vi "shearview_v1_0_oscillatoryshear__bfb7da842b.vi"() -> ()   [LabVIEW 2023]
uses:
  <instrlib>/niDCPower/nidcpower.llb/niDCPower Output Function.ctl
  <instrlib>/niDCPower/nidcpower.llb/niDCPower Source Mode.ctl
  <vilib>/Platform/TimedLoop/XDataNode/nitl_modes.ctl
  <vilib>/Platform/TimedLoop/XDataNode/timing_clust.ctl
  <vilib>/Platform/TimedLoop/XDataNode/wakeup.ctl
  <vilib>/Analysis/1siggen.llb/Ramp Pattern by Samples.vi
  <vilib>/DAQmx/create/channels.llb/DAQmx Create Channel (AI-Voltage-Basic).vi
  <vilib>/platform/TimedLoop/XDataNode/XDataNode.xnode
  <vilib>/Platform/TimedLoop/XDataNode/XDNodeRunTimeDep.lvlib
  <vilib>/Analysis/NI_AALBase.lvlib
panel:
  in  "stop 2":bool
  out "CPU Usage (%)":sgl(slide) scale=0.0..100.0
  out "Processor History":sgl(graph)
  in  "Tab Control 2":T1(tab)
  in  "Title of experiment":string="Shear Profiles " caption="A"
  in  "User":string="Nikos" caption="A"
  in  "Keywords":string caption="A"
  in  "Description":string="Profiles" caption="A"
  in  "Sample":string caption="A"
  in  "Temperature (oC)":string="23" caption="A"
  in  "Objective:":string="ELWD x20 " caption="A"
  in  "Numerical Aperture":string="0.45" caption="A"
  in  "Phase Annulus":string="Ph 1" caption="A"
  in  "Camera":string="Ximea MC050MG-SY-UB" caption="A"
  in  "Binning":string="2x2" caption="A"
  in  "Frame Rate (fps)":string="100 " caption="A"
  out "Finished Late? [i-1]":bool
  out "Iteration Duration":i64 format="%.2f"
  in  "Gap (mm)":dbl=1.0
  in  "Initial position in Voltage (V)":dbl=3.8
  in  "Voltage to Displacement Constant (V/mm)":dbl=0.689
  in  "Strain (%)":dbl=100.0
  in  "Frequency (Hz)":dbl=1.0 format="%0.3f"
  out "Elapsedf time (s)":dbl
  in  "samples":i32=7
  in  "end":dbl=100.0 format="%0.2f"
  in  "start":dbl=10.0 format="%0.2f"
  out "Ramp Pattern":dbl[](array[numeric])
  in  "type":u16(ring)=1 items=["Linear", "Logarithmic"]
  out "amplitude":dbl
  out "PID called time (s)":dbl format="%.3f"
  in  "Initial PID gains":T2={"proportional gain (Kc)"=0.1, "integral time (Ti, min)"=0.01, "derivative time (Td, min)"=0.0} {"derivative time (Td, min)" format="%.5f"; "integral time (Ti, min)" format="%.5f"; "proportional gain (Kc)" format="%.3f"}
  in  "PID dt (s)":dbl=0.003 format="%.3f"
  in  "Output current limit":dbl(slide)=0.49999999999999994 scale=0.0..1.0
  in  "Propotional":dbl(slide)=0.3411214953271028 scale=0.0..1.0
  in  "Integral":dbl(slide)=0.0002102803738317757 scale=0.0..0.0002
  in  "Derivative":dbl(slide) scale=0.0..0.001
  out "task done?":bool
  out "mean strain (-)":dbl
  out "min strain (-)":dbl
  out "max strain (-)":dbl
  out "mean current(A)":dbl
  in  "frames/period":dbl=12.0
  in  "offset (sec)":dbl=0.005
  in  "Exposure (s)  2":dbl=0.0001
  in  "Frequency":dbl=100.0 format="%.6f"
  in  "Duty Cycle":dbl=0.01 format="%.6f"
  in  "Number of Pulses":i32=1000
  in  "Imaging Selection":enum16{"No Imaging", "Profiles", "Echoes"}(ring)
  out "output array":cluster{dbl, dbl}[](array[cluster])
  out "error out":errorcluster
  out "Error":errorcluster
  out "error out 2":errorcluster
  in  "Tab Control":enum32{"Lissajous", "Strain-Stress"}(tab)
  out "?":cluster{dbl[], dbl[]}(graph)
  out "Mixed Signal Graph 5":dynamicdata(graph) caption="Commanded and Actual Strain vs Current"
  out "Queue timed out?":bool
  in  "stop":bool
  in  "stop initial loop":bool
  in  "file path":path=path "C:/Users/PC/Desktop/Data/tests/test.txt"
  # "Control Loop"
  # "Control Loop  Output"
  # "Parameters of Echoes"
  # "Parameters of Profiles"
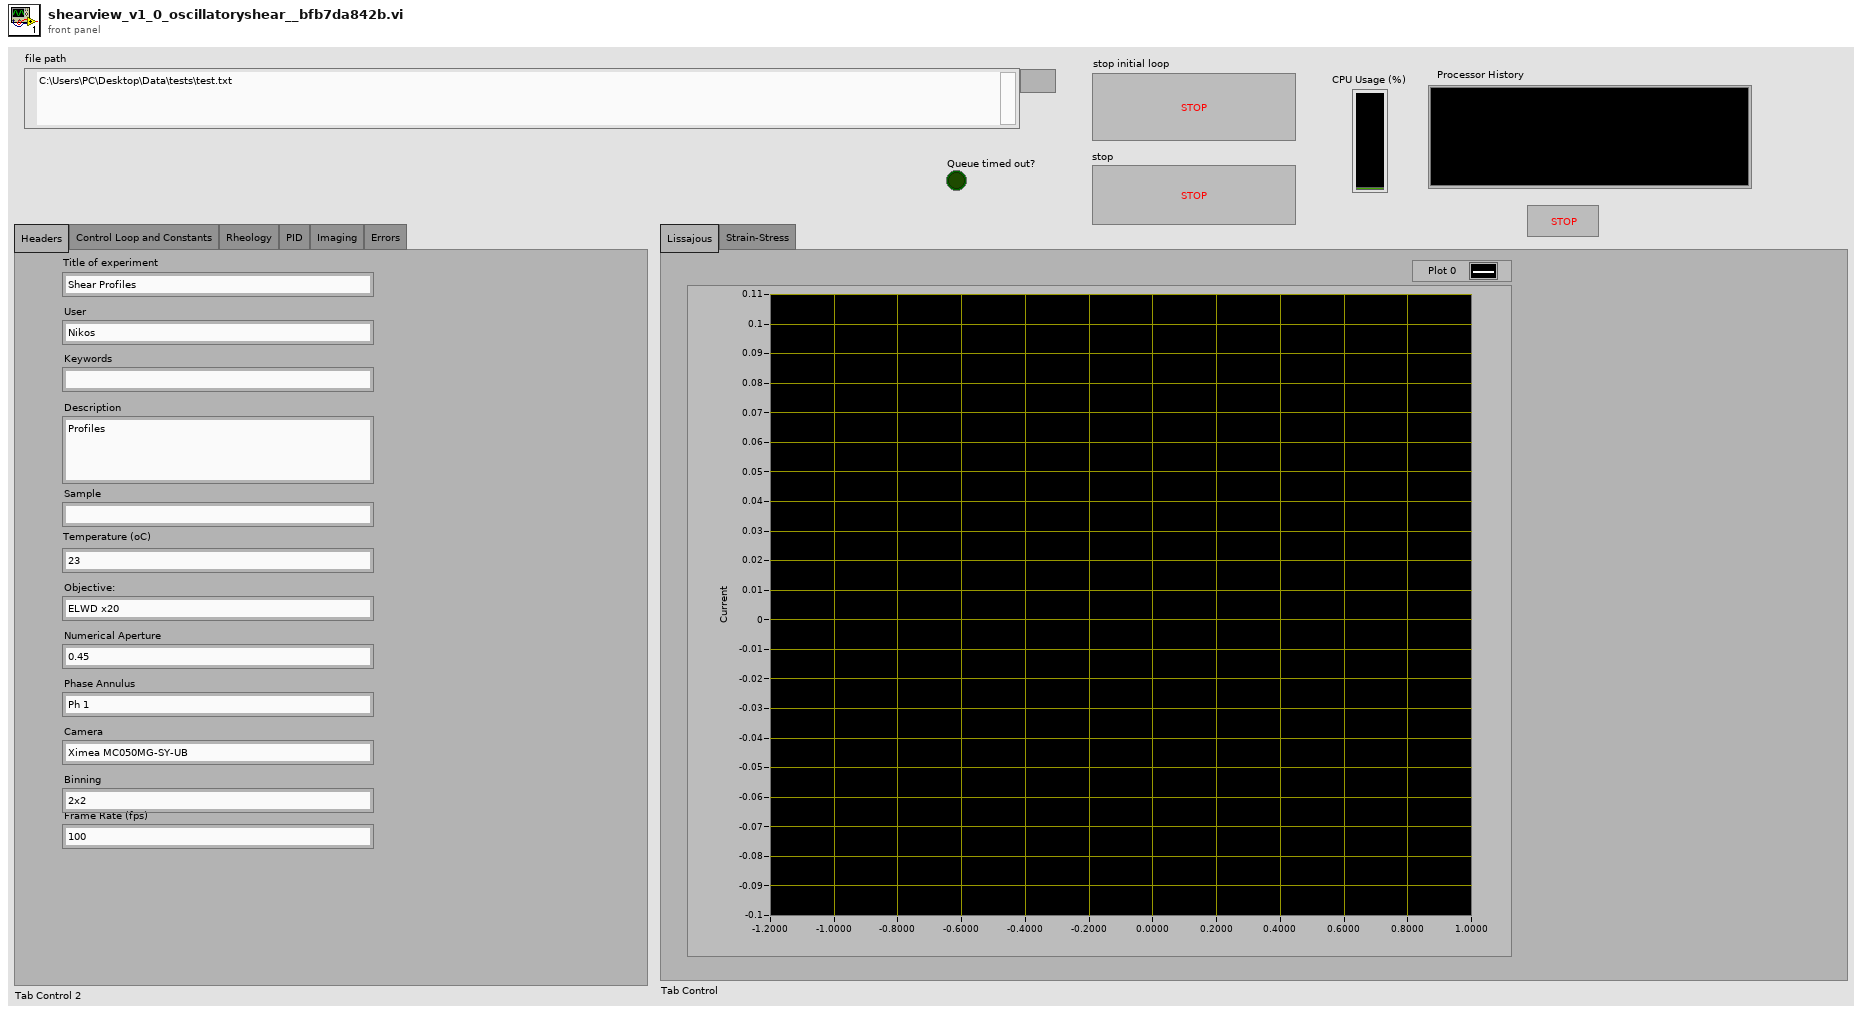
[diagram p1: front panel]
types:
  T1 = enum32{"Headers", "Control Loop and Constants", "Rheology", "PID", "Imaging", "Errors"}
  T2 = cluster{"proportional gain (Kc)":dbl, "integral time (Ti, min)":dbl, "derivative time (Td, min)":dbl}
  T3 = typedef "niDCPower Source Mode.ctl" = i32
  T4 = typedef "niDCPower Output Function.ctl" = i32
  T5 = typedef "XDNodeRunTimeDep.lvlib/nitl_modes.ctl" = enum32{"No Change", "Process missed periods, maintain original phase", "Discard missed periods, maintain original phase", "Process missed periods, ignore original phase", "Discard missed periods, ignore original phase"}
  T6 = typedef "XDNodeRunTimeDep.lvlib/timing_clust.ctl" = cluster{"Expected End [f-1]":u64, "Actual End [f-1]":u64, "Finished Late? [f-1]":bool, "Expected End [i-1]":u64, "Actual End [i-1]":u64, "Finished Late? [i-1]":bool, "Expected Start [i]":u64, "Actual Start [i]":u64, "Expected Start [f]":u64, "Actual Start [f]":u64, "Source Name":string, "Structure Name":string, "Period":i64, "Deadline":i64, "Offset":i64, "Start":i64, "Priority":i32, "Timeout":i32, "Mode":T5, "Wakeup Reason":T7, "Error":errorcluster, "Source Type":string, "Secondary Source Type":string, "Global End Time":u64, "Global Start Time":u64, "Frame Duration":u64, "Iteration Duration":u64, "Assigned CPU":i32, "I/O Scan Engine Mode":u32}
  T7 = typedef "XDNodeRunTimeDep.lvlib/wakeup.ctl" = enum32{"Normal", "Aborted", "Asynchronous wakeup", "Timing source error", "Timed loop error", "Timeout"}
  T8 = cluster{"time":dbl, "data":dbl, "set point":dbl, "time stress":dbl, "voltage":dbl, "current":dbl}
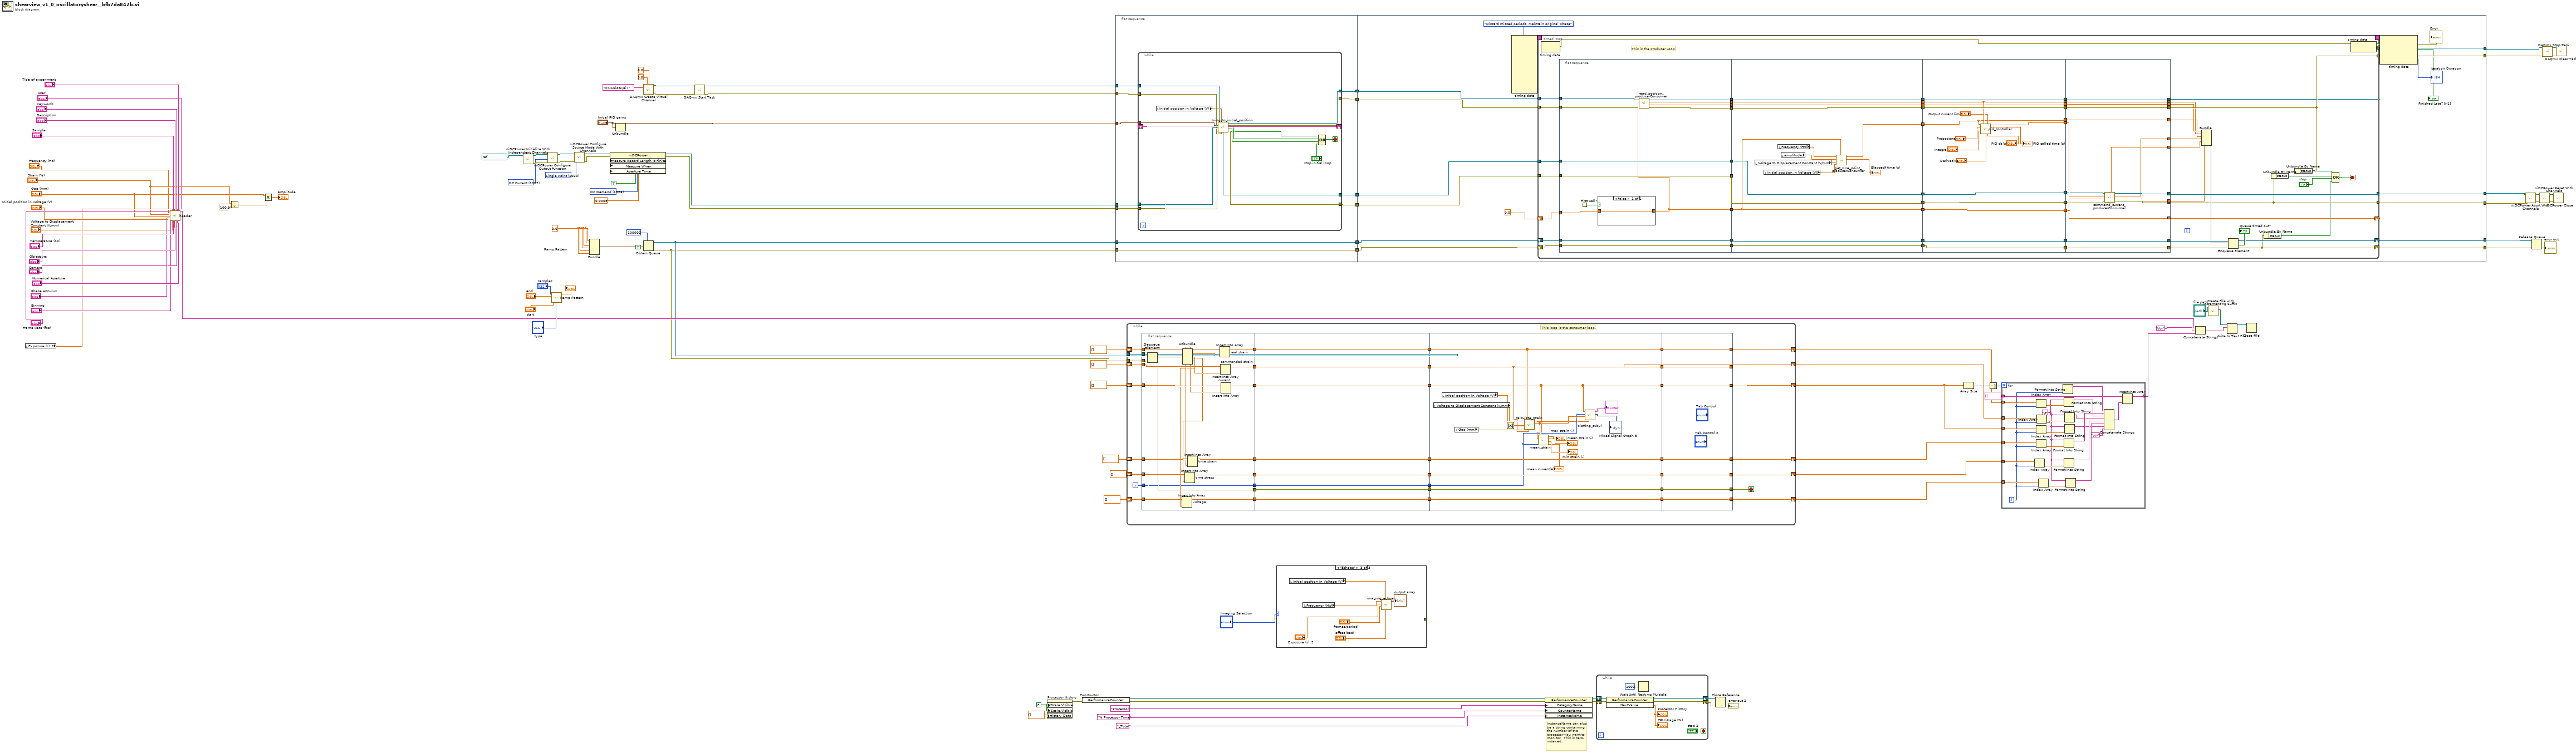
[diagram p0: block diagram]
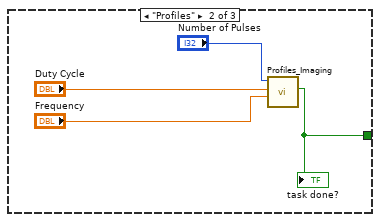
[diagram p3: hidden frame]
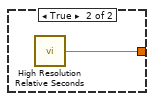
[diagram p4: hidden frame]
diagram:
  w7 = FALSE ("X Scale.Visible")
  w27 = 0.0
  w65 = T3 1020 items=["Single Point"=1020, "Sequence"=1021] ("source mode")
  w95 = 1026 items=["Automatically after Source Complete"=1025, "On Demand"=1026, "On Measure Trigger"=1027] ("Measurement:Advanced:Measure When")
  w101 = T4 1007 items=["DC Voltage"=1006, "DC Current"=1007, "Pulse Voltage"=1049, "Pulse Current"=1050] ("output function")
  # "InstanceName can also\nbe a string containing\nthe number of the\nprocessor you want to\nmonitor.  This is zero-\nindexed."
  n1 = local read "Exposure (s)  2"() -> (w45:dbl)
  n2 = call "header.vi"("Frequency (Hz)"="Frequency (Hz)", "Frame Rate (fps)"="Frame Rate (fps)", "Strain (%)"="Strain (%)", "Binning"="Binning", "Gap (mm)"="Gap (mm)", "Phase Annulus"="Phase Annulus", "Initial position in Voltage (V)"="Initial position in Voltage (V)", "Exposure (s)"=w45, "Voltage to Displacement Constant (V/mm)"="Voltage to Displacement Constant (V/mm)", "Sample"="Sample", "Temperature (oC)"="Temperature (oC)", "Description"="Description", "Objective:"="Objective:", "Keywords"="Keywords", "Camera"="Camera", "User"="User", "Numerical Aperture"="Numerical Aperture", "Title of experiment"="Title of experiment") -> ("String"=w44:string)  [unwired: 9 in]
  n3 = Divide(x="Strain (%)", y=100.0) -> (x/y=w43:dbl)
  n4 = Multiply(x="Gap (mm)", y=w43) -> (x*y=→"amplitude":dbl)
  n5 = call <instrlib>:"niDCPower Initialize With Independent Channels.vi"("resource name"=refnum<k15> "PXI1Slot3") -> ("error out"=w103:errorcluster, "instrument handle out"=w102:refnum<k15>)  [unwired: 9 in]
  n6 = call <instrlib>:"niDCPower Configure Output Function.vi"("error in (no error)"=w103, "output function"=w101, "instrument handle"=w102) -> ("error out"=w99:errorcluster, "instrument handle out"=w100:refnum<k15>)  [unwired: 7 in]
  n7 = call-poly <vilib>:"Ramp Pattern.vi"("type"="type", "start"="start", "end"="end", "samples"="samples") -> ("Ramp Pattern"=→"Ramp Pattern":dbl[])  [unwired: 6 in, 1 out]
  n8 = call <instrlib>:"niDCPower Configure Source Mode With Channels.vi"("error in (no error)"=w99, "source mode"=w65, "instrument handle"=w100) -> ("error out"=w91:errorcluster, "instrument handle out"=w90:refnum<k15>)  [unwired: 7 in]
  n9 = Bundle(w27, w27, w27, w27, w27, w27) -> (w28:cluster{dbl, dbl, dbl, dbl, dbl, dbl})  [unwired: 1 in]
  n10 = property class="niDCPower"(reference=w90, error in=w91, "Measure Record Length Is Finite"=TRUE ("Measurement:Measure Record Length Is Finite"), "Measure When"=w95, "Aperture Time"=0.0005 ("Measurement:Aperture Time")) -> (reference out=w73:refnum<k15>, error out=w94:errorcluster)
  n11 = Unbundle("Initial PID gains") -> ()  [unwired: 3 out]
  n12 = Obtain Queue(max queue size (-1, unlimited)=100000, element data type=w28, create if not found? (T)=TRUE) -> (queue out=w18:refnum<queue>, error out=w17:errorcluster)  [unwired: 2 in, 1 out]
  n13 = call-poly <vilib>:"DAQmx Create Virtual Channel.vi"("maximum value"=5.0, "minimum value"=0.0, "physical channels"=tag "PXI1Slot2/ai7") -> ("task out"=w86:refnum<k21>, "error out"=w85:errorcluster)  [unwired: 11 in]
  n14 = call <vilib>:"DAQmx Start Task.vi"("task/channels in"=w86, "error in"=w85) -> ("task out"=w106:refnum<k21>, "error out"=w66:errorcluster)  [unwired: 12 in]
  n15 = property on="Processor History" class="WFChart (strict)"("XScale.Visible"=w7, "YScale.Visible"=w7, "History Data"=sgl[] []) -> (error out=w4:errorcluster)  [unwired: 2 in, 1 out]
  n16 = constructor class="PerformanceCounter" ("Constructor Node")(error in=w4) -> (reference out=w16:refnum<k24>, error out=w15:errorcluster)  [unwired: 2 in, 1 out]
  n17 = flat-sequence {
    tunnel: w94 -> [w119]
    tunnel: w73 -> [w120]
    tunnel: w106 -> [w113]
    tunnel: [w117] -> w93
    tunnel: [w118] -> w92
    tunnel: "Initial PID gains" -> [w112]
    tunnel: [w116] -> w75
    tunnel: [w115] -> w74
    tunnel: w66 -> [w114]
    tunnel: [w111] -> w24
    tunnel: w18 -> [w111]
    tunnel: [w110] -> w23
    tunnel: w17 -> [w110]
    tunnel: [w154] -> w97
    tunnel: [w153] -> w3
    tunnel: w92 -> [w155]
    tunnel: w93 -> [w156]
    tunnel: [w138] -> w80
    tunnel: [w147] -> w79
    tunnel: w75 -> [w146]
    tunnel: w74 -> [w145]
    tunnel: [w142] -> w64
    tunnel: [w143] -> w63
    tunnel: w24 -> [w141]
    tunnel: w23 -> [w140]
    frame #0 {
      n18 = while {
        tunnel: [w137] -> w116
        tunnel: [w134] -> w115
        tunnel: w120 -> [w136]
        tunnel: w119 -> [w135]
        tunnel: [w133] -> w117
        tunnel: w113 -> [w124]
        tunnel: w114 -> [w123]
        tunnel: [w132] -> w118
        shift-right: [w131] -> _
        shift-left: _ -> [w130]
        tunnel: w112 -> [w122]
        stop <- w126 stop-if-true
        n19 = local read "Initial position in Voltage (V)"() -> (w121:dbl)
        n20 = call "bring_to_initial_position.vi"("Refnum in"=w124, "Initial position in Voltage (V) in"=w121, "Initial PID gains"=w122, "instrument handle in"=w136, "Array in"=w130, "error in (no error)"=w135, "error in"=w123) -> ("instrument handle out"=w132:refnum<k15>, "status"=w127:bool, "Refnum out"=w137:refnum<k21>, "error out 3"=w134:errorcluster, "status 2"=w128:bool, "Boolean"=w129:bool, "Array out"=w131:string[], "error out"=w133:errorcluster)  [unwired: 1 in]
        n21 = Compound Arithmetic op=OR(w127, w128, w129, "stop initial loop") -> (w126:bool)
      }
    }
    frame #1 {
      n22 = node-c288(nitl_modes."Discard missed periods, maintain original phase" ("Mode")) -> (w152:T6)  [unwired: 9 in]
      n23 = timed-loop {
        tunnel: w156 -> [w193]
        shift-right: [w177] -> _
        shift-left: 0.0 ("relative seconds") -> [w209]
        tunnel: w146 -> [w202]
        tunnel: w145 -> [w201]
        tunnel: w155 -> [w197]
        tunnel: [w191] -> w154
        tunnel: [w192] -> w153
        tunnel: [w189] -> w147
        timing: w152 -> [_]
        timing-out: [_] -> w151
        shift-right: [w161] -> w142
        shift-left: w141 -> [w184]
        shift-right: [w160] -> w143
        shift-left: w140 -> [w163]
        tunnel: [w157] -> w138
        stop <- w158 stop-if-true
        # "This is the Producer Loop"
        n24 = node-c288() -> (w188:errorcluster)  [unwired: 1 in]
        n25 = flat-sequence {
          tunnel: w202 -> [w232]
          tunnel: [w229] -> w216
          tunnel: [w234] -> w214
          tunnel: [w233] -> w211
          tunnel: w209 -> [w228]
          tunnel: w201 -> [w226]
          tunnel: [w231] -> w198
          tunnel: w197 -> [w231]
          tunnel: [w230] -> w194
          tunnel: w193 -> [w230]
          tunnel: [w227] -> w190
          tunnel: w184 -> [w224]
          tunnel: [w224] -> w183
          tunnel: [w223] -> w176
          tunnel: [w222] -> w164
          tunnel: w163 -> [w222]
          tunnel: w216 -> [w251]
          tunnel: [w251] -> w215
          tunnel: w214 -> [w250]
          tunnel: [w250] -> w213
          tunnel: [w247] -> w212
          tunnel: w211 -> [w248]
          tunnel: [w248] -> w210
          tunnel: [w237] -> w208
          tunnel: [w249] -> w199
          tunnel: w198 -> [w249]
          tunnel: [w245] -> w195
          tunnel: w194 -> [w245]
          tunnel: w190 -> [w237]
          tunnel: w183 -> [w244]
          tunnel: [w244] -> w181
          tunnel: w176 -> [w243]
          tunnel: [w243] -> w175
          tunnel: w164 -> [w238]
          tunnel: [w238] -> w162
          tunnel: w215 -> [w264]
          tunnel: w213 -> [w268]
          tunnel: w212 -> [w253]
          tunnel: w210 -> [w263]
          tunnel: w208 -> [w267]
          tunnel: [w264] -> w207
          tunnel: [w268] -> w206
          tunnel: [w263] -> w205
          tunnel: [w256] -> w204
          tunnel: [w267] -> w203
          tunnel: [w265] -> w200
          tunnel: w199 -> [w265]
          tunnel: [w266] -> w196
          tunnel: w195 -> [w266]
          tunnel: [w255] -> w182
          tunnel: w181 -> [w255]
          tunnel: [w252] -> w178
          tunnel: w175 -> [w254]
          tunnel: [w254] -> w174
          tunnel: [w253] -> w172
          tunnel: w162 -> [w252]
          tunnel: [w278] -> w177
          tunnel: [w282] -> w167
          tunnel: [w283] -> w192
          tunnel: [w284] -> w191
          tunnel: w207 -> [w284]
          tunnel: w206 -> [w283]
          tunnel: w205 -> [w282]
          tunnel: w204 -> [w281]
          tunnel: w203 -> [w278]
          tunnel: w200 -> [w277]
          tunnel: w196 -> [w280]
          tunnel: [w279] -> w157
          tunnel: [w276] -> w189
          tunnel: [w275] -> w180
          tunnel: w182 -> [w275]
          tunnel: [w274] -> w179
          tunnel: w178 -> [w274]
          tunnel: w174 -> [w273]
          tunnel: [w273] -> w173
          tunnel: [w272] -> w166
          tunnel: w172 -> [w272]
          tunnel: [w271] -> w171
          tunnel: [w270] -> w170
          tunnel: [w269] -> w169
          frame #0 {
            n26 = First Call?() -> (First Call?: T/F=w225:bool)
            n27 = case shown="False" w225 {
              tunnel: [w235 w236] -> w227
              tunnel: w228 -> [w235 _]
              frame False {
              }
              frame True {
                n28 = call <vilib>:"High Resolution Relative Seconds.vi"() -> ("relative seconds"=w236:dbl)
              }
            }
            n29 = call "read_position_producerConsumer.vi"("error in (no error)"=w226, "relative seconds"=w227, "Refnum in"=w232) -> ("error out"=w234:errorcluster, "time"=w223:dbl, "data"=w233:dbl, "Refnum out"=w229:refnum<k21>)  [unwired: 5 in]
          }
          frame #1 {
            n30 = local read "Voltage to Displacement Constant (V/mm)"() -> (w240:dbl)
            n31 = local read "Initial position in Voltage (V)"() -> (w239:dbl)
            n32 = local read "Frequency (Hz)"() -> (w242:dbl)
            n33 = local read "amplitude"() -> (w241:dbl)
            n34 = call "get_sine_point_producerConsumer.vi"("relative seconds"=w237, "Initial position in voltage"=w239, "voltage to displacement constant"=w240, "amplitude"=w241, "frequency"=w242) -> ("Elapsedf time (s)"=→"Elapsedf time (s)":dbl, "set point"=w247:dbl)  [unwired: 5 in]
          }
          frame #2 {
            n35 = call "pid_controller.vi"("set point"=w253, "process variable"=w263, "Output current limit"="Output current limit", "Propotional"="Propotional", "Integral"="Integral", "Derivative"="Derivative", "PID dt (s)"="PID dt (s)") -> ("output"=w256:dbl, "PID called time (s)"=→"PID called time (s)":dbl)  [unwired: 7 in]
          }
          frame #3 {
            n36 = call "command_current_producerConsumer.vi"("error in (no error)"=w280, "relative seconds"=w278, "PID output"=w281, "IVI Refnum in"=w277) -> ("error out"=w279:errorcluster, "time stress"=w271:dbl, "IVI Refnum out"=w276:refnum<k15>, "current"=w269:dbl, "voltage"=w270:dbl)  [unwired: 3 in]
          }
        }
        n37 = Bundle("time"=w173, "data"=w167, "set point"=w166, "time stress"=w171, "voltage"=w170, "current"=w169) -> (w168:T8)  [unwired: 1 in]
        n38 = Enqueue Element(queue=w180, element=w168, error in (no error)=w179) -> (queue out=w161:refnum<queue>, timed out?=→"Queue timed out?":bool, error out=w160:errorcluster)  [unwired: 1 in]
        n39 = Unbundle By Name(w160) -> ("status"=w159:bool)
        n40 = Unbundle By Name(w157) -> ("status"=w186:bool)
        n41 = Unbundle By Name(w192) -> ("status"=w187:bool)
        n42 = Compound Arithmetic op=OR(w187, w186, "stop", w159) -> (w158:bool)
        n43 = node-c288(w188) -> ()  [unwired: 1 out]
      }
      n44 = node-c288(w151) -> (→"Error":errorcluster, →"Finished Late? [i-1]":bool, →"Iteration Duration":i64)  [unwired: 1 out]
    }
  }
  n45 = while {
    tunnel: w18 -> [w330]
    shift-right: [w328] -> w22
    shift-left: dbl[] [] -> [w329]
    shift-right: [w327] -> w34
    shift-left: dbl[] [] -> [w326]
    shift-right: [w325] -> w33
    shift-left: dbl[] [] -> [w324]
    shift-right: [w322] -> w35
    shift-left: dbl[] [] -> [w323]
    shift-right: [w319] -> w31
    shift-left: dbl[] [] -> [w320]
    shift-right: [w321] -> w32
    shift-left: dbl[] [] -> [w318]
    tunnel: w17 -> [w317]
    i -> [w293]
    stop <- w296 stop-if-true
    # "This loop is the consumer loop."
    n46 = flat-sequence {
      tunnel: w330 -> [w353]
      tunnel: w329 -> [w351]
      tunnel: w326 -> [w348]
      tunnel: w324 -> [w346]
      tunnel: w323 -> [w345]
      tunnel: w320 -> [w342]
      tunnel: w318 -> [w340]
      tunnel: w317 -> [w339]
      tunnel: [w350] -> w316
      tunnel: [w349] -> w315
      tunnel: [w347] -> w314
      tunnel: [w344] -> w313
      tunnel: [w343] -> w312
      tunnel: [w341] -> w311
      tunnel: [w332] -> w298
      tunnel: [w331] -> w294
      tunnel: w293 -> [w331]
      tunnel: w316 -> [w361]
      tunnel: w315 -> [w360]
      tunnel: w314 -> [w359]
      tunnel: w313 -> [w358]
      tunnel: w312 -> [w357]
      tunnel: w311 -> [w356]
      tunnel: [w361] -> w310
      tunnel: [w360] -> w309
      tunnel: [w359] -> w308
      tunnel: [w358] -> w307
      tunnel: [w357] -> w306
      tunnel: [w356] -> w305
      tunnel: w298 -> [w355]
      tunnel: [w355] -> w297
      tunnel: w294 -> [w354]
      tunnel: [w354] -> w292
      tunnel: w310 -> [w367]
      tunnel: w309 -> [w366]
      tunnel: w308 -> [w362]
      tunnel: w307 -> [w381]
      tunnel: w306 -> [w380]
      tunnel: w305 -> [w379]
      tunnel: [w367] -> w304
      tunnel: [w366] -> w303
      tunnel: [w362] -> w302
      tunnel: [w381] -> w301
      tunnel: [w380] -> w300
      tunnel: [w379] -> w299
      tunnel: w297 -> [w368]
      tunnel: [w368] -> w295
      tunnel: w292 -> [w365]
      tunnel: [w383] -> w319
      tunnel: [w384] -> w321
      tunnel: [w385] -> w322
      tunnel: [w386] -> w325
      tunnel: [w387] -> w327
      tunnel: [w388] -> w328
      tunnel: w304 -> [w388]
      tunnel: w303 -> [w387]
      tunnel: w302 -> [w386]
      tunnel: w301 -> [w385]
      tunnel: w300 -> [w384]
      tunnel: w299 -> [w383]
      tunnel: [w382] -> w296
      tunnel: w295 -> [w382]
      frame #0 {
        n47 = Dequeue Element(queue=w353, error in (no error)=w339) -> (element=w352:cluster{dbl, dbl, dbl, dbl, dbl, dbl}, error out=w332:errorcluster)  [unwired: 1 in, 2 out]
        n48 = Unbundle(w352) -> (w335:dbl, w338:dbl, w337:dbl, w334:dbl, w333:dbl, w336:dbl)
        n49 = Insert Into Array "voltage"(array=w342, new element=w333) -> (w341:dbl[])  [unwired: 1 in]
        n50 = Insert Into Array "time stress"(array=w340, new element=w334) -> (w343:dbl[])  [unwired: 1 in]
        n51 = Insert Into Array "time strain"(array=w345, new element=w335) -> (w344:dbl[])  [unwired: 1 in]
        n52 = Insert Into Array "real strain"(array=w351, new element=w338) -> (w350:dbl[])  [unwired: 1 in]
        n53 = Insert Into Array "commanded strain"(array=w348, new element=w337) -> (w349:dbl[])  [unwired: 1 in]
        n54 = Insert Into Array "current"(array=w346, new element=w336) -> (w347:dbl[])  [unwired: 1 in]
      }
      frame #1 {
      }
      frame #2 {
        n55 = local read "Voltage to Displacement Constant (V/mm)"() -> (w376:dbl)
        n56 = local read "Initial position in Voltage (V)"() -> (w378:dbl)
        n57 = local read "Gap (mm)"() -> (w377:dbl)
        n58 = Absolute Value(x=w376) -> (abs(x)=w375:dbl)
        n59 = call "calculate_strain.vi"("commanded strain"=w366, "real strain"=w367, "Gap"=w377, "voltage to displacement contant"=w375, "initial position in volt"=w378) -> ("real strain (-)"=w374:dbl[], "commanded strain (-)"=w364:dbl[])  [unwired: 5 in]
        n60 = call "mean_strain.vi"("Iteration"=w365, "current"=w362, "real strain"=w374) -> ("mean current(A)"=→"mean current(A)":dbl, "min strain (-)"=→"min strain (-)":dbl, "mean strain (-)"=→"mean strain (-)":dbl, "max strain (-)"=→"max strain (-)":dbl)  [unwired: 3 in, 2 out]
        n61 = call "plotting_subvi.vi"("commanded strain"=w364, "real strain (-)"=w374, "iteration"=w365, "current"=w362) -> ("Mixed Signal Graph"=→"Mixed Signal Graph 5":dynamicdata, "Lissajou"=→"?":cluster{dbl[], dbl[]})  [unwired: 6 in]
      }
      frame #3 {
      }
    }
  }
  n62 = case shown="\"Echoes\"" "Imaging Selection" {
    tunnel: [_ w392 _] -> _
    frame "No Imaging" {
    }
    frame "Profiles" {
      n63 = call "Profiles_Imaging.vi"("Frequency"="Frequency", "Duty Cycle"="Duty Cycle", "Number of Pulses"="Number of Pulses") -> ("task done?"=w392:bool)  [unwired: 8 in]
      "task done?" <- w392
    }
    frame "Echoes" {
      n64 = local read "Initial position in Voltage (V)"() -> (w394:dbl)
      n65 = local read "Frequency (Hz)"() -> (w395:dbl)
      n66 = call "imaging_echoes.vi"("offset (sec)"="offset (sec)", "trigger voltage"=w394, "frames/period"="frames/period", "Exposure (s)"="Exposure (s)  2", "frequency"=w395) -> ("output array"=→"output array":cluster{dbl, dbl}[])  [unwired: 6 in]
    }
  }
  n67 = property on="Property Node" class="PerformanceCounter"(reference=w16, error in=w15, "CategoryName"="Processor", "CounterName"="% Processor Time", "InstanceName"="_Total") -> (reference out=w12:refnum<k24>, error out=w11:errorcluster)
  n68 = while {
    shift-right: [w402] -> w9
    shift-left: w12 -> [w405]
    shift-right: [w403] -> w10
    shift-left: w11 -> [w404]
    stop <- "stop 2" stop-if-true
    n69 = invoke on="Invoke Node" class="PerformanceCounter" method="NextValue"(reference=w405, error in=w404) -> (reference out=w402:refnum<k24>, error out=w403:errorcluster, "NextValue"=→"CPU Usage (%)" →"Processor History":sgl)  [unwired: 1 in]
    n70 = Wait Until Next ms Multiple(millisecond multiple=u32 1000 ("milliseconds to wait")) -> ()  [unwired: 1 out]
  }
  n71 = Close Reference(reference=w9, error in (no error)=w10) -> (error out=→"error out 2":errorcluster)
  n72 = Array Size(array=w33) -> (size(s)=w20:i32)
  n73 = Decrement(x=w20) -> (x-1=w19:i32)
  n74 = for {
    N: w19 -> [_]
    tunnel: w35 -> [w419]
    tunnel: w34 -> [w415]
    tunnel: w33 -> [w417]
    tunnel: w32 -> [w421]
    tunnel: w31 -> [w407]
    tunnel: w22 -> [w423]
    tunnel: string[] [] -> [w409]
    tunnel: [w410] -> w30 mode=concatenating
    i -> [w406]
    w412 = "\t"
    n75 = Index Array(array=w421, index=w406) -> (element=w420:dbl)
    n76 = Index Array(array=w423, index=w406) -> (element=w424:dbl)
    n77 = Index Array(array=w417, index=w406) -> (element=w416:dbl)
    n78 = Index Array(array=w419, index=w406) -> (element=w418:dbl)
    n79 = Index Array(array=w415, index=w406) -> (element=w414:dbl)
    n80 = Index Array(array=w407, index=w406) -> (element=w422:dbl)
    n81 = Format Into String(w406) -> (resulting string=w413:string)  [unwired: 3 in, 1 out]
    n82 = Format Into String(initial string=w412, w424) -> (resulting string=w429:string)  [unwired: 2 in, 1 out]
    n83 = Format Into String(initial string=w412, w418) -> (resulting string=w430:string)  [unwired: 2 in, 1 out]
    n84 = Format Into String(initial string=w412, w420) -> (resulting string=w427:string)  [unwired: 2 in, 1 out]
    n85 = Format Into String(initial string=w412, w414) -> (resulting string=w428:string)  [unwired: 2 in, 1 out]
    n86 = Format Into String(initial string=w412, w416) -> (resulting string=w425:string)  [unwired: 2 in, 1 out]
    n87 = Format Into String(initial string=w412, w422) -> (resulting string=w426:string)  [unwired: 2 in, 1 out]
    n88 = Concatenate Strings(w413, w430, w429, w428, w427, w426, w425, "\r\n") -> (w411:string)
    n89 = Insert Into Array(array=w409, new element=w411) -> (w410:string[])  [unwired: 1 in]
  }
  n90 = Concatenate Strings(w44, "\r\n", w30) -> (w87:string)
  n91 = call <vilib>:"Create File with Incrementing Suffix.vi"("file path"="file path") -> ("actual path"=w77:path)  [unwired: 8 in, 2 out]
  n92 = Write to Text File(file (use dialog)=w77, text=w87) -> (refnum out=w89:refnum<file>)  [unwired: 2 in, 2 out]
  n93 = Close File(refnum=w89) -> ()  [unwired: 1 in, 2 out]
  n94 = call <instrlib>:"niDCPower Abort With Channels.vi"("error in (no error)"=w80, "instrument handle"=w79) -> ("error out"=w81:errorcluster, "instrument handle out"=w82:refnum<k15>)  [unwired: 8 in]
  n95 = Release Queue(queue=w64, error in (no error)=w63) -> (error out=→"error out":errorcluster)  [unwired: 1 in, 2 out]
  n96 = call <instrlib>:"niDCPower Reset With Channels.vi"("error in (no error)"=w81, "instrument handle"=w82) -> ("error out"=w83:errorcluster, "instrument handle out"=w84:refnum<k15>)  [unwired: 8 in]
  n97 = call <vilib>:"DAQmx Stop Task.vi"("task/channels in"=w97, "error in"=w3) -> ("task out"=w105:refnum<k21>, "error out"=w104:errorcluster)  [unwired: 12 in]
  n98 = call <instrlib>:"niDCPower Close.vi"("error in (no error)"=w83, "instrument handle"=w84) -> ()  [unwired: 9 in, 1 out]
  n99 = call <vilib>:"DAQmx Clear Task.vi"("task in"=w105, "error in"=w104) -> ()  [unwired: 13 in, 1 out]
